vi "Main Test.vi"() -> ()   [LabVIEW 2023]
uses:
  <extravilib>/ChannelInstances/Tag-bool.lvlib
  DUT Sample/typedefs/DO Finite Pulse Config.ctl
  DUT Sample/DUT Sample.lvclass
  DUT Sample/typedefs/Signal Value.ctl
panel:
  in  "Command DO Pulse":bool
  out "error out":errorcluster
  in  "stop":bool
  out "Array":T1[](array[typedef])
  in  "Intf.CAN.Term":bool=TRUE
  in  "DO Finite Pulse Config":T2={"Port Number"=0, "Number of Pulses"=20, "High Time (ms)"=20, "Low Time (ms)"=20}
  in  "Write Data":bool
  in  "Intf.BaudRate64":u64=500000
  in  "signal list to read":refnum<k21>[](array[refnum])=["Error_Active\nHW_Val_CAN_DUT_Sample", "Error_Code\nHW_Val_CAN_DUT_Sample", "Pulse_Success\nHW_Val_CAN_DUT_Sample", "DO_Pulse_Done.DO_Port\nHW_Val_CAN_DUT_Sample"]
  in  "interface":refnum<k21>
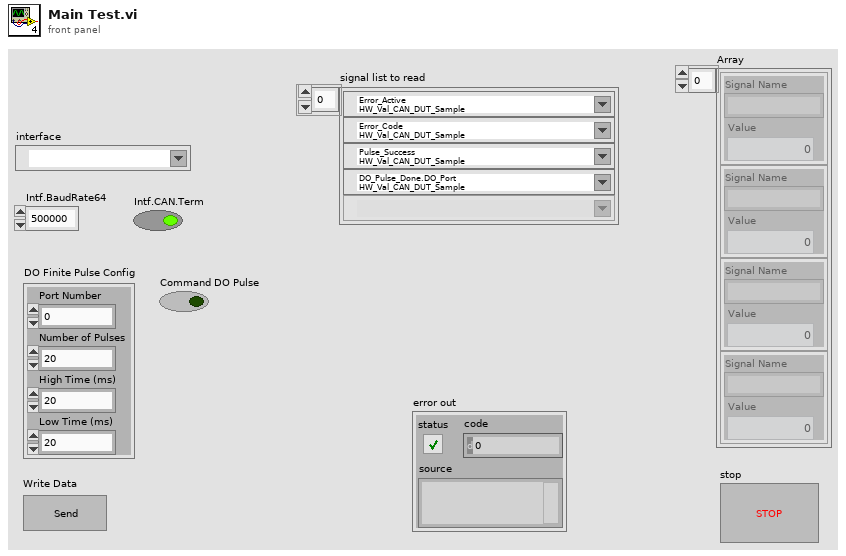
[diagram p1: front panel]
types:
  T1 = typedef "Signal Value.ctl" = cluster{"Signal Name":string, "Value":dbl}
  T2 = typedef "DUT Sample.lvclass/DO Finite Pulse Config.ctl" = cluster{"Port Number":u8, "Number of Pulses":u8, "High Time (ms)":u16, "Low Time (ms)":u16}
  T3 = typedef "Tag-bool.lvlib/))Channel.ctl" = refnum<queue>
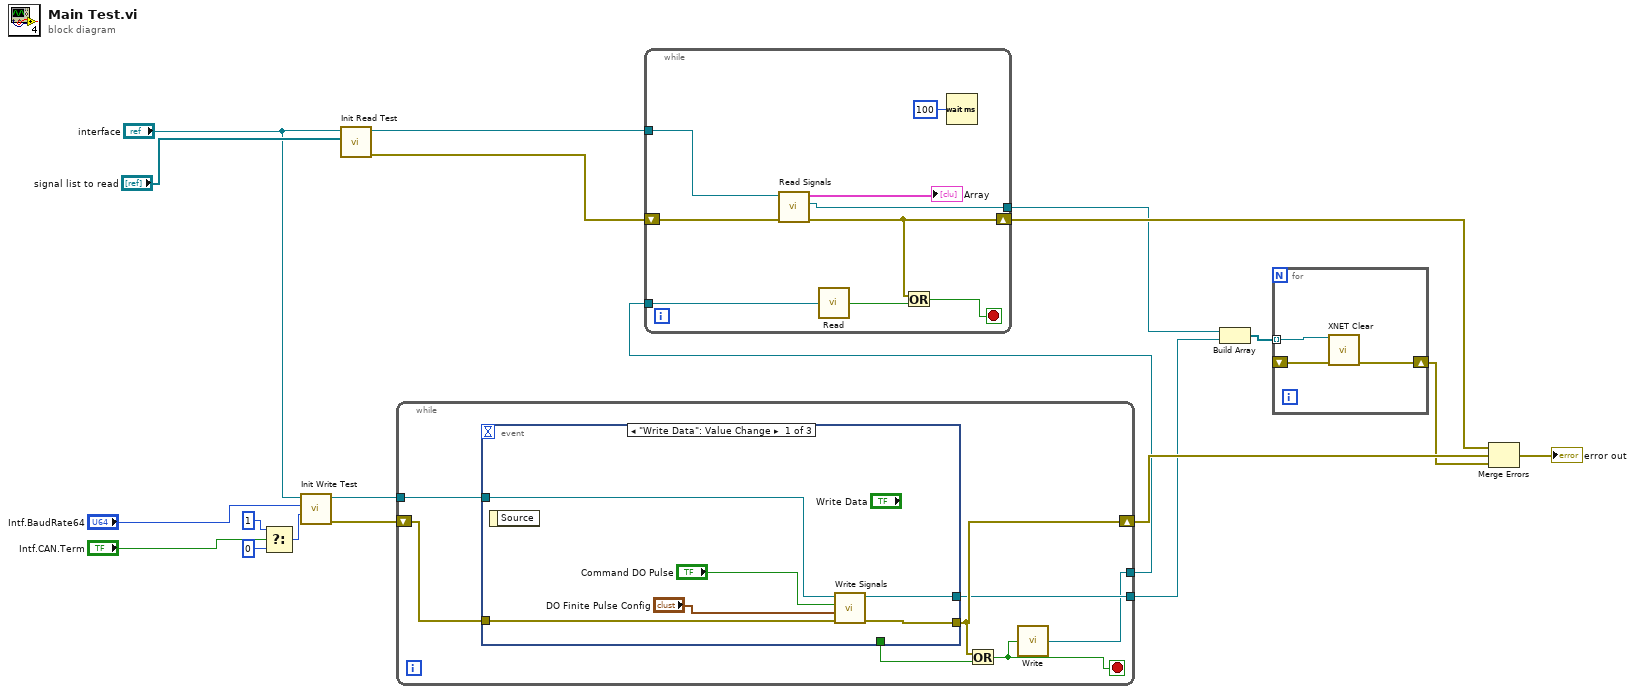
[diagram p0: block diagram]
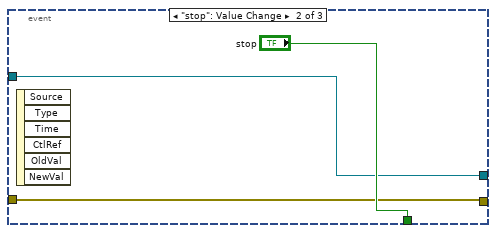
[diagram p2: hidden frame]
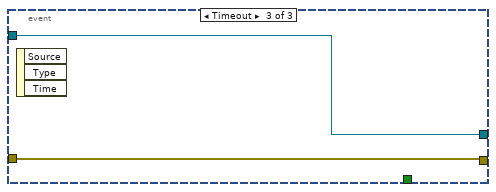
[diagram p3: hidden frame]
diagram:
  n1 = Select(t=1, s="Intf.CAN.Term", f=0) -> (s? t:f=w10:i32)
  n2 = call "Init Write Test.vi"("interface"="interface", "Intf.BaudRate64"="Intf.BaudRate64", "Intf.CAN.Term"=w10) -> ("session out"=w14:refnum<k21>, "error out"=w13:errorcluster)  [unwired: 6 in]
  n3 = call "Init Read Test.vi"("signal list"="signal list to read", "interface"="interface") -> ("error out"=w15:errorcluster, "session out"=w16:refnum<k21>)  [unwired: 8 in]
  n4 = while {
    tunnel: w14 -> [w20]
    shift-right: [w25] -> w9
    shift-left: w13 -> [w26]
    tunnel: [w24] -> w5
    tunnel: [w21] -> w2
    stop <- w22 stop-if-true
    n5 = event shown="[0] \"Write Data\": Value Change" {
      selector: _ -> [_ _ _]
      dyn-events: _ -> [_ _ _]
      timeout: _ -> [_ _ _]
      tunnel: w26 -> [w32 w33 w37]
      tunnel: [w31 w33 w37] -> w25
      tunnel: [w30 w34 w36] -> w24
      tunnel: [_ "stop" _] -> w23
      tunnel: w20 -> [w29 w34 w36]
      event "Write Data": Value Change {
        n6 = event-data() -> ()  [unwired: 1 in, 1 out]
        n7 = call "Write Signals.vi"("error in (no error)"=w32, "DO Finite Pulse Config"="DO Finite Pulse Config", "Command DO Pulse"="Command DO Pulse", "session in"=w29) -> ("error out"=w31:errorcluster, "session out"=w30:refnum<k21>)  [unwired: 6 in]
      }
      event "stop": Value Change {
        n8 = event-data() -> ()  [unwired: 1 in, 6 out]
      }
      event Timeout {
        n9 = event-data() -> ()  [unwired: 1 in, 3 out]
      }
    }
    n10 = Or(x=w25, y=w23) -> (x .or. y?=w22:bool)
    n11 = call <extravilib>:"Write.vi"("element"=w22) -> ("channel"=w21:T3)  [unwired: 1 out]
  }
  n12 = while {
    tunnel: w16 -> [w46]
    shift-right: [w40] -> w8
    shift-left: w15 -> [w45]
    tunnel: w2 -> [w42]
    tunnel: [w39] -> w6
    stop <- w43 stop-if-true
    n13 = call "Read Signals.vi"("error in (no error)"=w45, "session in"=w46) -> ("error out"=w40:errorcluster, "session out"=w39:refnum<k21>, "Array"=→"Array":T1[])  [unwired: 7 in]
    n14 = call <extravilib>:"Read.vi"("channel"=w42) -> ("element"=w41:bool)  [unwired: 1 in, 1 out]
    n15 = Or(x=w40, y=w41) -> (x .or. y?=w43:bool)
    n16 = Wait (ms)(milliseconds to wait=u32 100) -> ()  [unwired: 1 out]
  }
  n17 = Build Array(w6, w5) -> (w4:refnum<k21>[])
  n18 = for {
    tunnel: w4 -> [w49] mode=indexing
    shift-right: [w48] -> w3
    shift-left: _ -> [w47]
    n19 = call <vilib>:"XNET Clear.vi"("session in"=w49, "error in (no error)"=w47) -> ("error out"=w48:errorcluster)  [unwired: 13 in]
  }
  n20 = Merge Errors(w8, w9, w3) -> (→"error out":errorcluster)
